vi "ArmTuningPathGenerator.vi"() -> (4 "Rotation Motion Profile":T2[](array[typedef]) {"Time (ms)" items=["TrajectoryDuration_0ms"=0, "TrajectoryDuration_5ms"=5, "TrajectoryDuration_10ms"=10, "TrajectoryDuration_20ms"=20, "TrajectoryDuration_30ms"=30, "TrajectoryDuration_40ms"=40, "TrajectoryDuration_50ms"=50, "TrajectoryDuration_100ms"=100]}, 6 "Extension Motion Profile":T2[](array[typedef]) {"Time (ms)" items=["TrajectoryDuration_0ms"=0, "TrajectoryDuration_5ms"=5, "TrajectoryDuration_10ms"=10, "TrajectoryDuration_20ms"=20, "TrajectoryDuration_30ms"=30, "TrajectoryDuration_40ms"=40, "TrajectoryDuration_50ms"=50, "TrajectoryDuration_100ms"=100]}, 8 "Go":bool)   [LabVIEW 2017]
uses:
  General/MotionProfiling/TypeDefs/MotionProfileGeneratorParams.ctl
  <vilib>/Rock Robotics/WPI/ThirdParty/Phoenix-LabVIEW/Motor Controller/Controls/CTRE_Phoenix_MotorControl_TrajectoryPointTimeDur.ctl
  General/MotionProfiling/TypeDefs/TrajectoryPoint.ctl
  ArgosLib/Signal Processing/TypeDefs/EdgeDetector_Type.ctl
  ArgosLib/ArgosLib.lvlib
panel:
  in  "Enable extension":bool
  in  "Enable rotation":bool
  out "Extension Motion Profile Graph":T1(graph)
  out "Rotation Motion Profile Graph":T1(graph)
  in  "MotionProfileGeneratorParameters":T4={"Trajectory Point Interval (ms)"=10, "Maximum Travel Speed (units/s)"=500.0, "Velocity Ramp Time (ms)"=400.0, "Acceleration Ramp Time (ms)"=200.0} {"Acceleration Ramp Time (ms)" min=1.0; "Velocity Ramp Time (ms)" min=1.0; "Maximum Travel Speed (units/s)" min=0.0; "Trajectory Point Interval (ms)" items=["TrajectoryDuration_0ms"=0, "TrajectoryDuration_5ms"=5, "TrajectoryDuration_10ms"=10, "TrajectoryDuration_20ms"=20, "TrajectoryDuration_30ms"=30, "TrajectoryDuration_40ms"=40, "TrajectoryDuration_50ms"=50, "TrajectoryDuration_100ms"=100]}
  in  "Reverse Direction":bool
  in  "Send Motion Profiles":bool
  in  "End Extension":dbl
  in  "Start Extension":dbl
  in  "End Angle":dbl
  in  "Start Angle":dbl
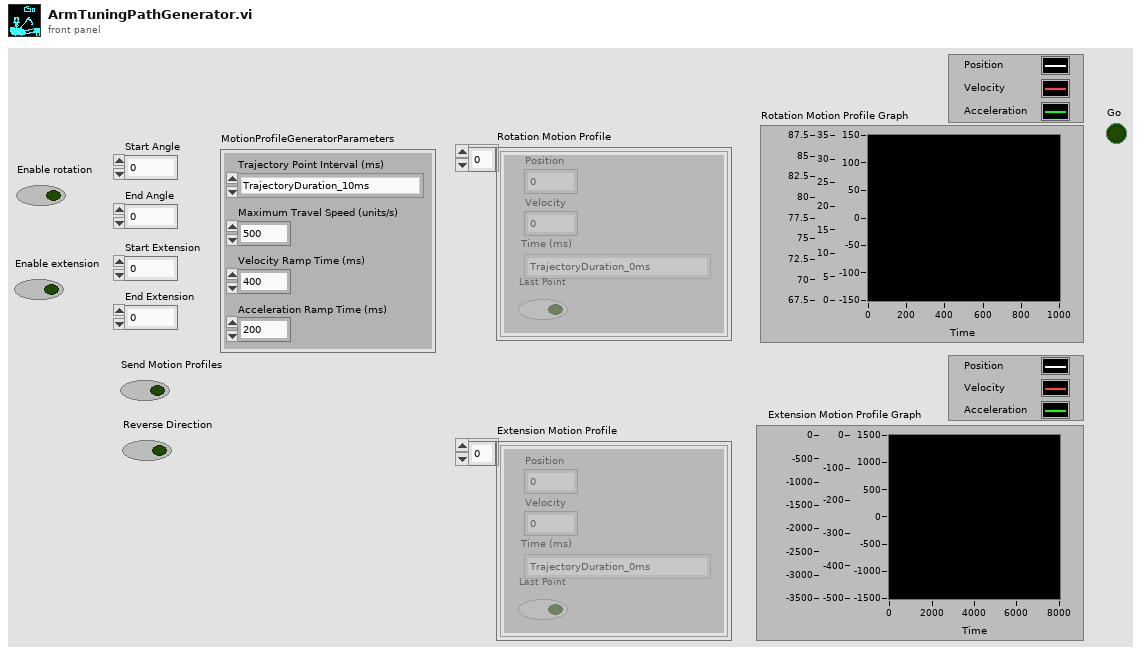
[diagram p1: front panel]
types:
  T1 = cluster{dbl, "Trajectory Point Interval (ms)":i32, dbl[][]}
  T2 = typedef "TrajectoryPoint.ctl" = cluster{"Position ":dbl, "Velocity ":dbl, "Time (ms)":T3, "Last Point":bool}
  T3 = typedef "CTRE_Phoenix_MotorControl_TrajectoryPointTimeDur.ctl" = i32
  T4 = typedef "MotionProfileGeneratorParams.ctl" = cluster{"Trajectory Point Interval (ms)":T3, "Maximum Travel Speed (units/s)":dbl, "Velocity Ramp Time (ms)":dbl, "Acceleration Ramp Time (ms)":dbl}
  T5 = typedef "ArgosLib.lvlib/EdgeDetector_Type.ctl" = enum16{"RisingEdge", "FallingEdge", "Both"}
  T6 = cluster{dbl, "Trajectory Point Interval (ms)":T3, dbl[][]}
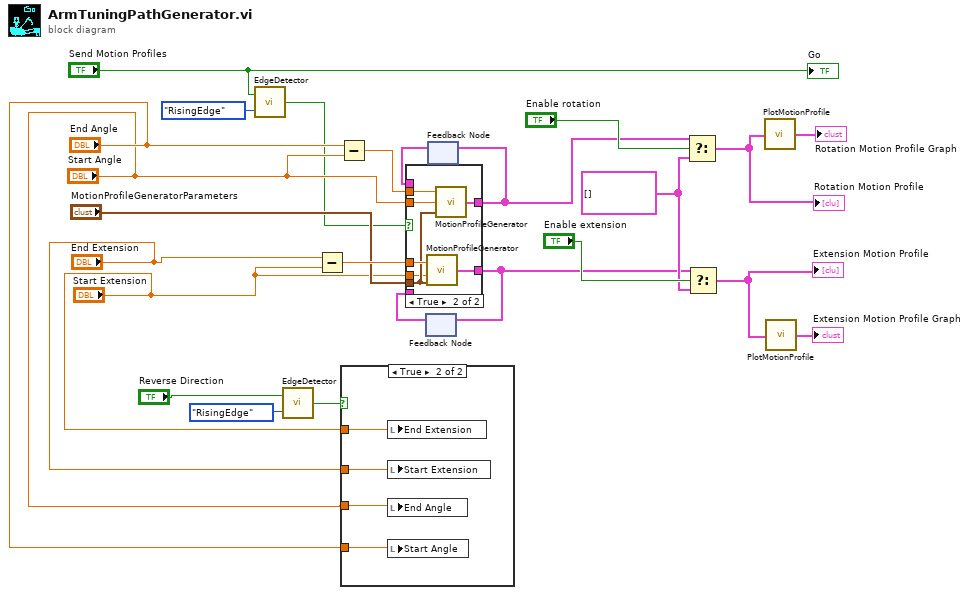
[diagram p0: block diagram]
diagram:
  w8 = T2[] [] ("f")
  n1 = call "EdgeDetector.vi"("DetectorType"=EdgeDetector_Type."RisingEdge", "Input"="Send Motion Profiles") -> ("Edge"=w3:bool)
  n2 = call "EdgeDetector.vi"("DetectorType"=EdgeDetector_Type."RisingEdge", "Input"="Reverse Direction") -> ("Edge"=w16:bool)
  n3 = Subtract(x="End Extension", y="Start Extension") -> (x-y=w23:dbl)
  n4 = Subtract(x="End Angle", y="Start Angle") -> (x-y=w24:dbl)
  n5 = case shown="True" w16 {
    tunnel: "End Angle" -> [_ w28]
    tunnel: "Start Angle" -> [_ w27]
    tunnel: "End Extension" -> [_ w26]
    tunnel: "Start Extension" -> [_ w25]
    frame False {
    }
    frame True {
      n6 = local write "End Extension"(w25) -> ()
      n7 = local write "Start Extension"(w26) -> ()
      n8 = local write "End Angle"(w27) -> ()
      n9 = local write "Start Angle"(w28) -> ()
    }
  }
  n10 = feedback #1() -> (w6:T2[])  [unwired: 1 in]
  n11 = feedback #2() -> (w4:T2[])  [unwired: 1 in]
  n12 = case shown="True" w3 {
    tunnel: w24 -> [_ w37]
    tunnel: w23 -> [_ w36]
    tunnel: "MotionProfileGeneratorParameters" -> [_ w35]
    tunnel: "Start Extension" -> [_ w34]
    tunnel: "Start Angle" -> [_ w33]
    tunnel: [w29 w32] -> w5
    tunnel: [w30 w31] -> w7
    tunnel: w6 -> [w30 _]
    tunnel: w4 -> [w29 _]
    frame False {
    }
    frame True {
      n13 = call "MotionProfileGenerator.vi"("MotionProfileGeneratorParameters"=w35, "Starting Position (units)"=w34, "Travel Distance (units)"=w36) -> ("Trajectory Points"=w31:T2[])
      n14 = call "MotionProfileGenerator.vi"("MotionProfileGeneratorParameters"=w35, "Starting Position (units)"=w33, "Travel Distance (units)"=w37) -> ("Trajectory Points"=w32:T2[])
    }
  }
  n15 = feedback-in #1(w7) -> ()
  n16 = feedback-in #2(w5) -> ()
  n17 = Select(t=w5, s="Enable rotation", f=w8) -> (s? t:f=w9:T2[])
  "Rotation Motion Profile" <- w9
  n18 = Select(t=w7, s="Enable extension", f=w8) -> (s? t:f=w10:T2[])
  "Extension Motion Profile" <- w10
  n19 = call "PlotMotionProfile.vi"("Trajectory Points"=w9) -> ("MotionProfileGraph"=→"Rotation Motion Profile Graph":T6)
  n20 = call "PlotMotionProfile.vi"("Trajectory Points"=w10) -> ("MotionProfileGraph"=→"Extension Motion Profile Graph":T6)
  "Go" <- "Send Motion Profiles"
